vi "Unqualify Item Name.vi"(11 "Item Name":string) -> (3 "Item Name out":string)   [LabVIEW 2020, in "VI Properties Editor.lvlib"]
doc: "Unqualifies <B>Item Name</B>, removing all namespacing."
uses:
  VI Properties Editor.lvlib
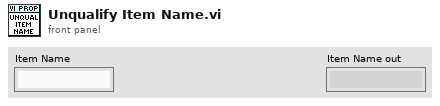
[diagram p1: front panel]
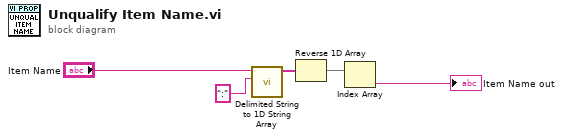
[diagram p0: block diagram]
diagram:
  n1 = call-poly <vilib>:"Delimited String to 1D String Array.vi"("delimiter"=":", "delimited string"="Item Name") -> ("string array"=w3:string[])  [unwired: 9 in]
  n2 = Reverse 1D Array(array=w3) -> (reversed array=w2:string[])
  n3 = Index Array(array=w2) -> (element=→"Item Name out":string)  [unwired: 1 in]
